vi "read_table_key_string.vi"(7 "table":string, 8 "error in (no error)":errorcluster, 9 "default (\"\")":string, 10 "key":string, 11 "toml in":refnum<class "toml.lvclass">) -> (0 "error out":errorcluster, 1 "value":string, 2 "found?":bool, 3 "toml out":refnum<class "toml.lvclass">)   [LabVIEW 2020, in "toml.lvclass"]
uses:
  toml.lvclass
  toml.lvclass/toml.ctl
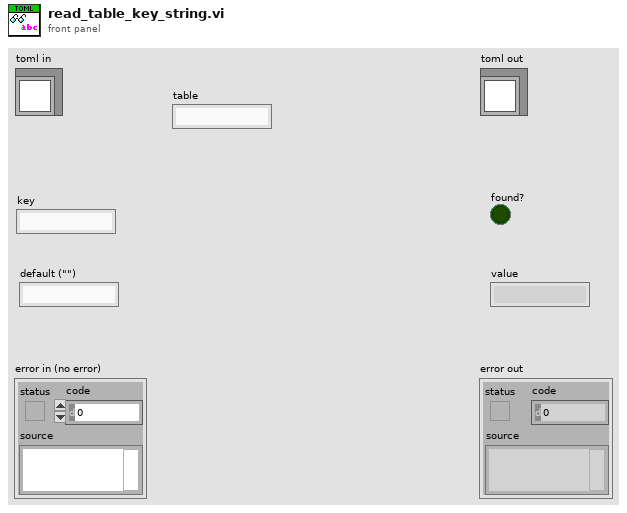
[diagram p1: front panel]
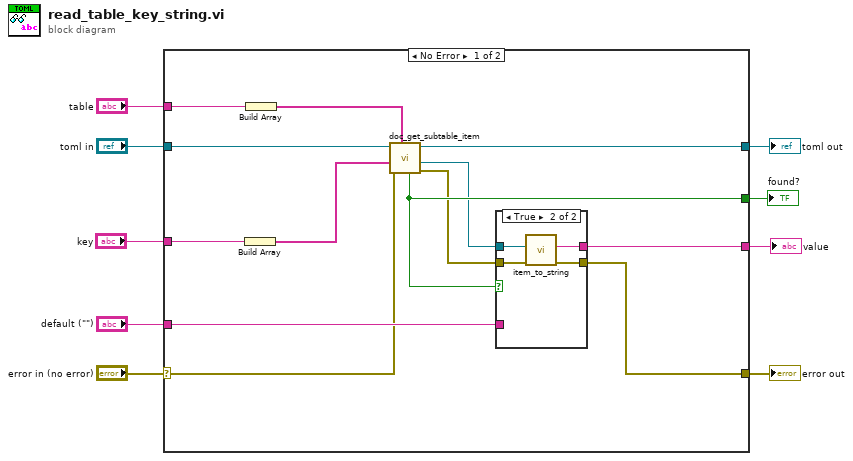
[diagram p0: block diagram]
diagram:
  n1 = case shown="No Error" "error in (no error)" {
    selector: "error in (no error)" -> [w18 w30]
    tunnel: [w19 w30] -> w8
    tunnel: [w10 w29] -> w6
    tunnel: "toml in" -> [w11 w29]
    tunnel: "table" -> [w22 _]
    tunnel: "key" -> [w21 _]
    tunnel: "default (\"\")" -> [w20 _]
    tunnel: [w17 _] -> w2
    tunnel: [w16 _] -> w1
    frame No Error {
      n2 = Build Array(w21) -> (w12:string[])
      n3 = Build Array(w22) -> (w15:string[])
      n4 = call "doc_get_subtable_item.vi"("subtables"=w15, "error in (no error)"=w18, "subkeys"=w12, "toml in"=w11) -> ("error out"=w13:errorcluster, "item (value)"=w14:refnum<class "Item.lvclass">, "toml out"=w10:refnum<class "toml.lvclass">, "found?"=w16:bool)  [unwired: 4 in]
      n5 = case shown="True" w16 {
        tunnel: w14 -> [_ w28]
        tunnel: [w24 w27] -> w17
        tunnel: w13 -> [w23 w26]
        tunnel: [w23 w25] -> w19
        tunnel: w20 -> [w24 _]
        frame False {
        }
        frame True {
          n6 = call "item_to_string.vi"("error in (no error)"=w26, "Item in"=w28) -> ("error out"=w25:errorcluster, "string_value"=w27:string)  [unwired: 8 in]
        }
      }
    }
    frame Error {
    }
  }
  "error out" <- w8
  "toml out" <- w6
  "value" <- w2
  "found?" <- w1
